vi "Raw to Signed Edge Case Tests.vi"() -> ()   [LabVIEW 2026, in "Utility.lvlib"]
doc: "Standalone test harness for signed-representation conversion. Replace placeholder actual result controls by wiring outputs from To Signed Representation.vim over each type test vector."
uses:
  Utility.lvlib
  Types/Signed Representation.ctl
  422b4465-0d46-49d9-81d2-ff2c9fbddcb7.vi
  29d09dfc-37e6-4d7c-9192-7f9a4cc0419b.vi
  8fd39e2a-21bd-4cbd-8027-f42b800c8f99.vi
  0e5b698d-5939-4f5d-b5fc-2d002ad3a321.vi
  422b4465-0d46-49d9-81d2-ff2c9fbddcb7.vi/075529c4-3756-4c35-a727-d79a570b4e4b.vi
  422b4465-0d46-49d9-81d2-ff2c9fbddcb7.vi/f2b159a7-3f15-4c07-8087-86d897f3e084.vi
  422b4465-0d46-49d9-81d2-ff2c9fbddcb7.vi/e7f4747e-5a28-4a2e-9592-f11bd74c8d05.vi
  422b4465-0d46-49d9-81d2-ff2c9fbddcb7.vi/dfb42b1f-79ab-4f7c-b389-1108b947dcfb.vi
  422b4465-0d46-49d9-81d2-ff2c9fbddcb7.vi/5f52ec6b-8d9c-4a1b-8cba-4e2f2acbbc65.vi
  422b4465-0d46-49d9-81d2-ff2c9fbddcb7.vi/9402299f-8d08-4b56-b955-c752433d99a7.vi
  422b4465-0d46-49d9-81d2-ff2c9fbddcb7.vi/587ca7da-2917-4b98-b856-e292118fa9d0.vi
  422b4465-0d46-49d9-81d2-ff2c9fbddcb7.vi/d9cf77ad-bfa9-4690-bb58-8188d63c027f.vi
  422b4465-0d46-49d9-81d2-ff2c9fbddcb7.vi/0dbe1b4e-815d-48eb-bf8e-9c4112dc030e.vi
  29d09dfc-37e6-4d7c-9192-7f9a4cc0419b.vi/075529c4-3756-4c35-a727-d79a570b4e4b.vi
  29d09dfc-37e6-4d7c-9192-7f9a4cc0419b.vi/f2b159a7-3f15-4c07-8087-86d897f3e084.vi
  29d09dfc-37e6-4d7c-9192-7f9a4cc0419b.vi/e7f4747e-5a28-4a2e-9592-f11bd74c8d05.vi
  29d09dfc-37e6-4d7c-9192-7f9a4cc0419b.vi/dfb42b1f-79ab-4f7c-b389-1108b947dcfb.vi
  29d09dfc-37e6-4d7c-9192-7f9a4cc0419b.vi/5f52ec6b-8d9c-4a1b-8cba-4e2f2acbbc65.vi
  29d09dfc-37e6-4d7c-9192-7f9a4cc0419b.vi/9402299f-8d08-4b56-b955-c752433d99a7.vi
  29d09dfc-37e6-4d7c-9192-7f9a4cc0419b.vi/587ca7da-2917-4b98-b856-e292118fa9d0.vi
  29d09dfc-37e6-4d7c-9192-7f9a4cc0419b.vi/d9cf77ad-bfa9-4690-bb58-8188d63c027f.vi
  29d09dfc-37e6-4d7c-9192-7f9a4cc0419b.vi/0dbe1b4e-815d-48eb-bf8e-9c4112dc030e.vi
  8fd39e2a-21bd-4cbd-8027-f42b800c8f99.vi/075529c4-3756-4c35-a727-d79a570b4e4b.vi
  8fd39e2a-21bd-4cbd-8027-f42b800c8f99.vi/f2b159a7-3f15-4c07-8087-86d897f3e084.vi
  8fd39e2a-21bd-4cbd-8027-f42b800c8f99.vi/e7f4747e-5a28-4a2e-9592-f11bd74c8d05.vi
  8fd39e2a-21bd-4cbd-8027-f42b800c8f99.vi/dfb42b1f-79ab-4f7c-b389-1108b947dcfb.vi
  8fd39e2a-21bd-4cbd-8027-f42b800c8f99.vi/5f52ec6b-8d9c-4a1b-8cba-4e2f2acbbc65.vi
  8fd39e2a-21bd-4cbd-8027-f42b800c8f99.vi/9402299f-8d08-4b56-b955-c752433d99a7.vi
  8fd39e2a-21bd-4cbd-8027-f42b800c8f99.vi/587ca7da-2917-4b98-b856-e292118fa9d0.vi
  8fd39e2a-21bd-4cbd-8027-f42b800c8f99.vi/d9cf77ad-bfa9-4690-bb58-8188d63c027f.vi
  8fd39e2a-21bd-4cbd-8027-f42b800c8f99.vi/0dbe1b4e-815d-48eb-bf8e-9c4112dc030e.vi
  0e5b698d-5939-4f5d-b5fc-2d002ad3a321.vi/075529c4-3756-4c35-a727-d79a570b4e4b.vi
  0e5b698d-5939-4f5d-b5fc-2d002ad3a321.vi/f2b159a7-3f15-4c07-8087-86d897f3e084.vi
  0e5b698d-5939-4f5d-b5fc-2d002ad3a321.vi/e7f4747e-5a28-4a2e-9592-f11bd74c8d05.vi
  0e5b698d-5939-4f5d-b5fc-2d002ad3a321.vi/dfb42b1f-79ab-4f7c-b389-1108b947dcfb.vi
  0e5b698d-5939-4f5d-b5fc-2d002ad3a321.vi/5f52ec6b-8d9c-4a1b-8cba-4e2f2acbbc65.vi
  0e5b698d-5939-4f5d-b5fc-2d002ad3a321.vi/9402299f-8d08-4b56-b955-c752433d99a7.vi
  0e5b698d-5939-4f5d-b5fc-2d002ad3a321.vi/587ca7da-2917-4b98-b856-e292118fa9d0.vi
  0e5b698d-5939-4f5d-b5fc-2d002ad3a321.vi/d9cf77ad-bfa9-4690-bb58-8188d63c027f.vi
  0e5b698d-5939-4f5d-b5fc-2d002ad3a321.vi/0dbe1b4e-815d-48eb-bf8e-9c4112dc030e.vi
panel:
  in  "i64 expected encoded":i64[](array[numeric])=[0, 0, 1, -1, 9223372036854775807, -9223372036854775807, 0, 0, 1, -1, 9223372036854775807, -9223372036854775807]
  in  "i32 expected encoded":i32[](array[numeric])=[0, 0, 1, -1, 2147483647, -2147483647, 0, 0, 1, -1, 2147483647, -2147483647]
  in  "i16 expected encoded":i16[](array[numeric])=[0, 0, 1, -1, 32767, -32767, 0, 0, 1, -1, 32767, -32767]
  in  "expected valid":bool[](array[boolean])=[TRUE, FALSE, TRUE, TRUE, TRUE, TRUE, TRUE, FALSE, TRUE, TRUE, TRUE, TRUE]
  in  "i8 expected":i8[](array[numeric])=[0, 0, 1, -1, 127, -127, 0, 0, 1, -1, 127, -127]
  out "all tests pass?":bool
  out "i64 pass?":bool
  in  "u64 test values":u64[](array[numeric])=[0, 9223372036854775808, 1, 9223372036854775809, 9223372036854775807, 18446744073709551615, 0, 18446744073709551615, 1, 18446744073709551614, 9223372036854775807, 9223372036854775808] format="%016x"
  out "i32 pass?":bool
  in  "u32 test values":u32[](array[numeric])=[0, 2147483648, 1, 2147483649, 2147483647, 4294967295, 0, 4294967295, 1, 4294967294, 2147483647, 2147483648] format="%08x"
  out "i16 pass?":bool
  in  "u16 test values":u16[](array[numeric])=[0, 32768, 1, 32769, 32767, 65535, 0, 65535, 1, 65534, 32767, 32768] format="%04x"
  out "i8 pass?":bool
  in  "test encodings":T1[](array[typedef])=[enum."Sign-Magnitude", enum."Sign-Magnitude", enum."Sign-Magnitude", enum."Sign-Magnitude", enum."Sign-Magnitude", enum."Sign-Magnitude", enum."Ones' Complement", enum."Ones' Complement", enum."Ones' Complement", enum."Ones' Complement", enum."Ones' Complement", enum."Ones' Complement"]
  in  "u8 test values":u8[](array[numeric])=[0, 128, 1, 129, 127, 255, 0, 255, 1, 254, 127, 128] format="%02x"
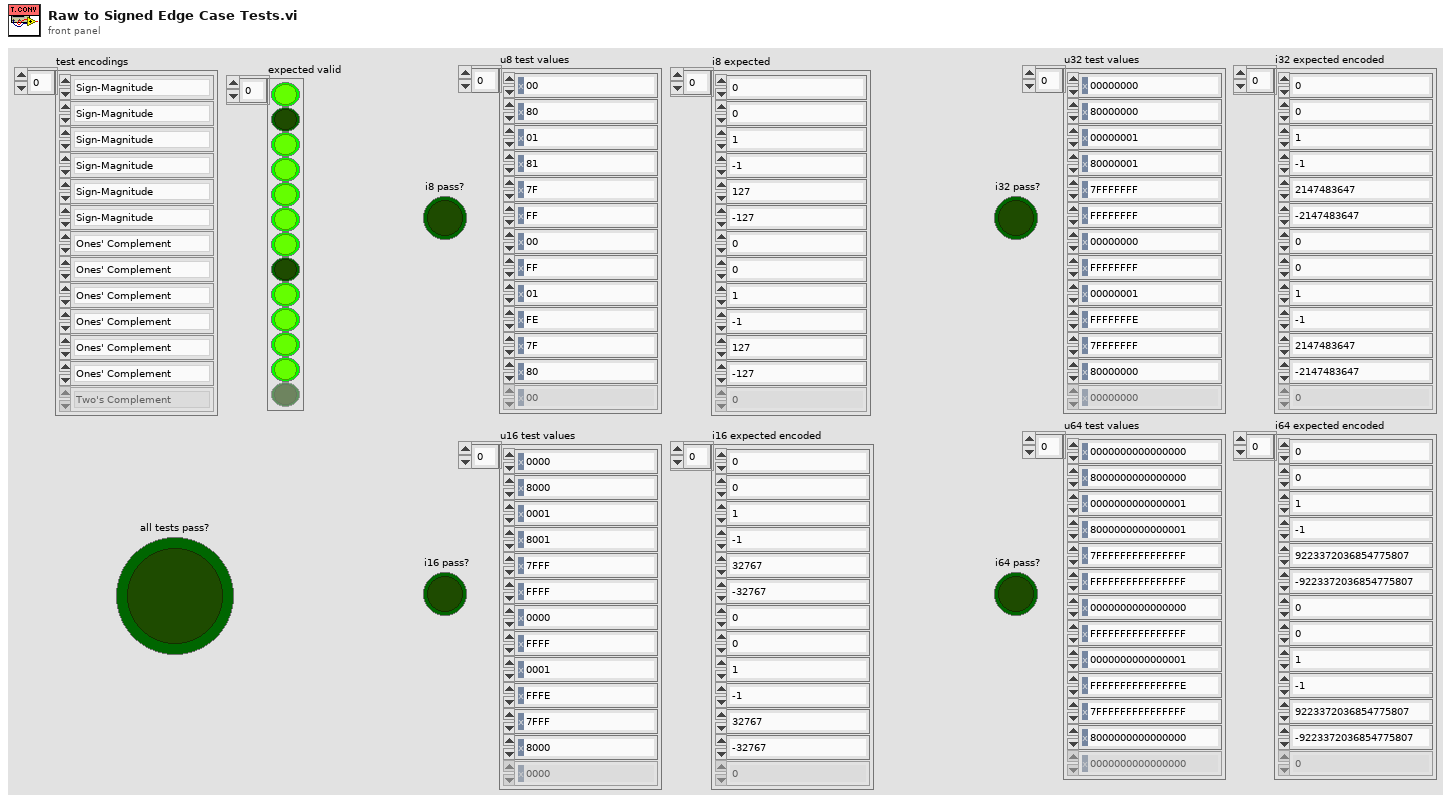
[diagram p1: front panel]
types:
  T1 = typedef "Utility.lvlib/Signed Representation.ctl" = enum16{"Two's Complement", "Offset Binary", "Sign-Magnitude", "Ones' Complement"}
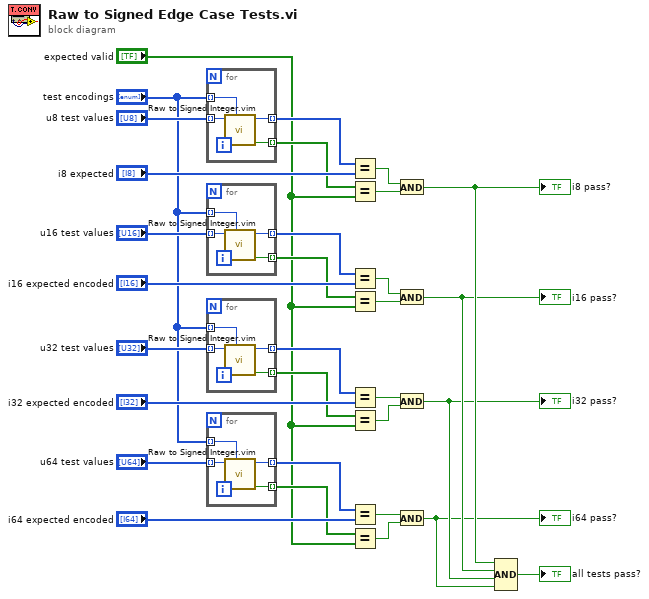
[diagram p0: block diagram]
diagram:
  n1 = for {
    tunnel: "test encodings" -> [w35] mode=indexing
    tunnel: "u8 test values" -> [w34] mode=indexing
    tunnel: [w33] -> w10 mode=indexing
    tunnel: [w32] -> w9 mode=indexing
    n2 = call "Raw to Signed Integer.vim"("Signed representation"=w35, "Value (raw)"=w34) -> ("Valid?"=w32:bool, "Value out"=w33:i8)  [unwired: 8 in]
  }
  n3 = for {
    tunnel: "test encodings" -> [w39] mode=indexing
    tunnel: "u16 test values" -> [w38] mode=indexing
    tunnel: [w37] -> w8 mode=indexing
    tunnel: [w36] -> w7 mode=indexing
    n4 = call "Raw to Signed Integer.vim"("Signed representation"=w39, "Value (raw)"=w38) -> ("Valid?"=w36:bool, "Value out"=w37:i16)  [unwired: 8 in]
  }
  n5 = for {
    tunnel: "test encodings" -> [w43] mode=indexing
    tunnel: "u32 test values" -> [w42] mode=indexing
    tunnel: [w41] -> w6 mode=indexing
    tunnel: [w40] -> w5 mode=indexing
    n6 = call "Raw to Signed Integer.vim"("Signed representation"=w43, "Value (raw)"=w42) -> ("Valid?"=w40:bool, "Value out"=w41:i32)  [unwired: 8 in]
  }
  n7 = for {
    tunnel: "test encodings" -> [w47] mode=indexing
    tunnel: "u64 test values" -> [w46] mode=indexing
    tunnel: [w45] -> w4 mode=indexing
    tunnel: [w44] -> w3 mode=indexing
    n8 = call "Raw to Signed Integer.vim"("Signed representation"=w47, "Value (raw)"=w46) -> ("Valid?"=w44:bool, "Value out"=w45:i64)  [unwired: 8 in]
  }
  n9 = Equal?(x=w10, y="i8 expected") -> (x = y?=w30:bool)
  n10 = Equal?(x=w9, y="expected valid") -> (x = y?=w29:bool)
  n11 = Equal?(x=w8, y="i16 expected encoded") -> (x = y?=w27:bool)
  n12 = Equal?(x=w7, y="expected valid") -> (x = y?=w26:bool)
  n13 = Equal?(x=w6, y="i32 expected encoded") -> (x = y?=w24:bool)
  n14 = Equal?(x=w5, y="expected valid") -> (x = y?=w23:bool)
  n15 = Equal?(x=w4, y="i64 expected encoded") -> (x = y?=w21:bool)
  n16 = Equal?(x=w3, y="expected valid") -> (x = y?=w20:bool)
  n17 = And(x=w30, y=w29) -> (x .and. y?=w18:bool)
  "i8 pass?" <- w18
  n18 = And(x=w27, y=w26) -> (x .and. y?=w17:bool)
  "i16 pass?" <- w17
  n19 = And(x=w24, y=w23) -> (x .and. y?=w16:bool)
  "i32 pass?" <- w16
  n20 = And(x=w21, y=w20) -> (x .and. y?=w15:bool)
  "i64 pass?" <- w15
  n21 = Compound Arithmetic op=AND(w18, w17, w16, w15) -> (→"all tests pass?":bool)
